vi "Labo03_NTC.vi"() -> ()   [LabVIEW 2021]
uses:
  <vilib>/express/express shared/transition.llb/Dynamic To Waveform Array.vi
  <vilib>/express/express arith-compare/Formula/Block/exnFormulaBlock how many pts in the wave.vi
  <vilib>/express/express shared/ex_Modify Signal Name.vi
  <vilib>/express/express shared/transition.llb/Waveform Array To Dynamic.vi
  <vilib>/express/express arith-compare/Formula/XNode/ExpressFormulaBlockNode.xnode
panel:
  out "Waveform Chart":dynamicdata(graph)
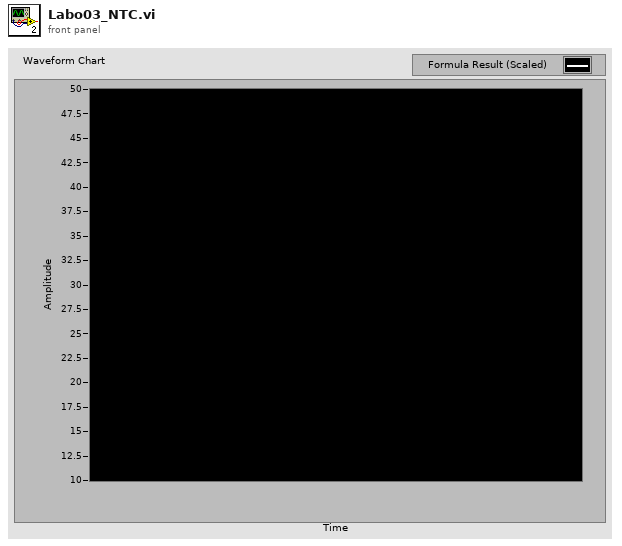
[diagram p1: front panel]
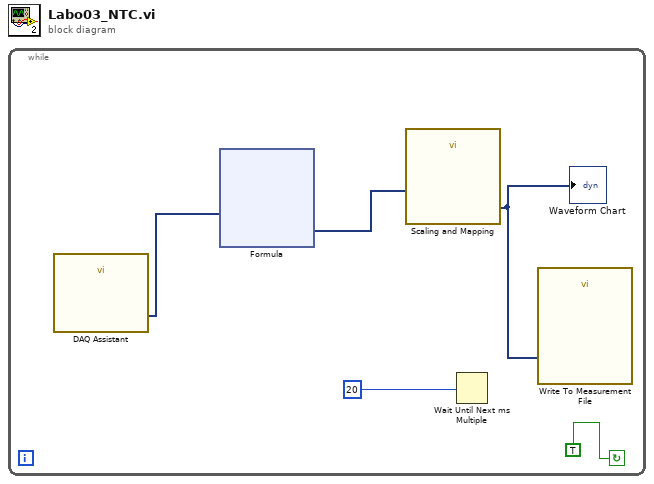
[diagram p0: block diagram]
diagram:
  n1 = while {
    stop <- TRUE continue-if-true
    n2 = call "DAQ Assistant"() -> ("data"=w2:dynamicdata)  [unwired: 17 in, 2 out]
    n3 = xnode "Formula"("X1"=w2) -> ("Result"=w5:dynamicdata)  [unwired: 1 in, 1 out]
    n4 = call "Scaling and Mapping"("Signals"=w5) -> ("Scaled Signals"=w1:dynamicdata)  [unwired: 9 in, 1 out]
    "Waveform Chart" <- w1
    n5 = Wait Until Next ms Multiple(millisecond multiple=20) -> ()  [unwired: 1 out]
    n6 = call "Write To Measurement File"("Signals"=w1) -> ()  [unwired: 16 in, 3 out]
  }
